vi "G4BaseTemplate_Singleton_5x6x5_CleanUp.vi"(11 "Error In":errorcluster) -> (15 "Error Out":errorcluster)   [LabVIEW 2020, in "G4BaseTemplate_Singleton_5x6x5.lvclass"]
uses:
  G4BaseTemplate_Singleton_5x6x5.lvclass
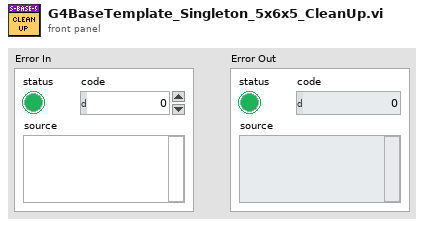
[diagram p1: front panel]
types:
  T1 = typedef "G4BaseTemplate_Singleton_5x6x5.lvclass/ObjectAttributes.ctl" = cluster{"Attribute1":dbl}
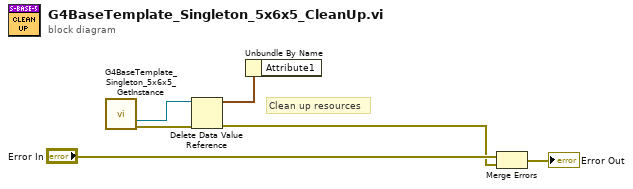
[diagram p0: block diagram]
diagram:
  # "Clean up resources"
  n1 = call "G4BaseTemplate_Singleton_5x6x5_GetInstance.vi"() -> ("DVRRefOut"=w2:refnum<data-value>, "Error Out"=w3:errorcluster)  [unwired: 11 in, 3 out]
  n2 = Delete Data Value Reference(data value reference=w2, error in=w3) -> (data value=w1:T1, error out=w4:errorcluster)
  n3 = Unbundle By Name(w1) -> ()  [unwired: 1 out]
  n4 = Merge Errors("Error In", w4) -> (→"Error Out":errorcluster)
